vi "RemoteVI Read Tips.vi"(0 "VI":refnum<vi>, 1 "refresh?":bool, 2 "origin":cluster{"x":i32, "y":i32}, 3 "message in":string="tips []", 5 "subpanels?":bool=TRUE) -> (4 "message out":string, 15 "error out":errorcluster)   [LabVIEW 2020, in "RemoteVI.lvlib"]
doc: "Reads the tip strips of the published panel for the tips message (docs\\protocol.md 3.3) - LabVIEW shows its own tip strips only while it is the foreground application, so the browser shows them itself. When refresh? is TRUE (the server loop just refreshed the geometry: every 500 ms, never while a popup or a modal window is open, because this is a VI Server call that would block in their modal loop), every visible control with a tip strip gives one entry: the controls RemoteVI Panel Controls.vi finds (top level of every pane, the selected page of a tab control, cluster elements, two levels deep) and those of a VI shown in a subpanel among them. An entry's bounds are the control's Position and Bounds (the label included) converted from its pane's coordinates to panel coordinates ({LV.Pane} CvtPaneToPanelCoords on the pane RemoteVI Panel Controls.vi gives; a subpanel VI's panes convert into the host panel), then to screen coordinates (CvtPanelToScreenCoords of the published panel), then to frame coordinates (minus the top-left of Front Panel Window:Panel Bounds, plus origin). Inner controls come first (subpanel VIs, then deeper levels), so the browser, which shows the first entry under the pointer, shows a cluster element's tip strip rather than its cluster's. RemoteVI Tips Message.vi builds message out from them. Otherwise, or on an error, message out is message in."
uses:
  RemoteVI.lvlib
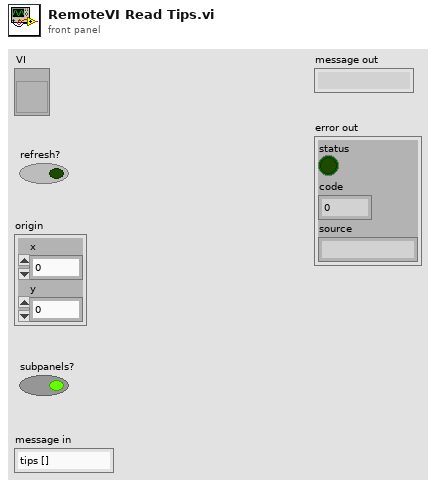
[diagram p1: front panel]
types:
  T1 = cluster{"x":i32, "y":i32, "w":i32, "h":i32, "text":string}
  T2 = typedef "LVRectTypeDef.ctl" = cluster{"left":i16, "top":i16, "right":i16, "bottom":i16}
  T3 = typedef "LVPositionTypeDef.ctl" = cluster{"Left":i32, "Top":i32}
  T4 = typedef "LVBoundsTypeDef.ctl" = cluster{"Width":u32, "Height":u32}
  T5 = typedef "LVPointTypeDef.ctl" = cluster{"Horizontal":i16, "Vertical":i16}
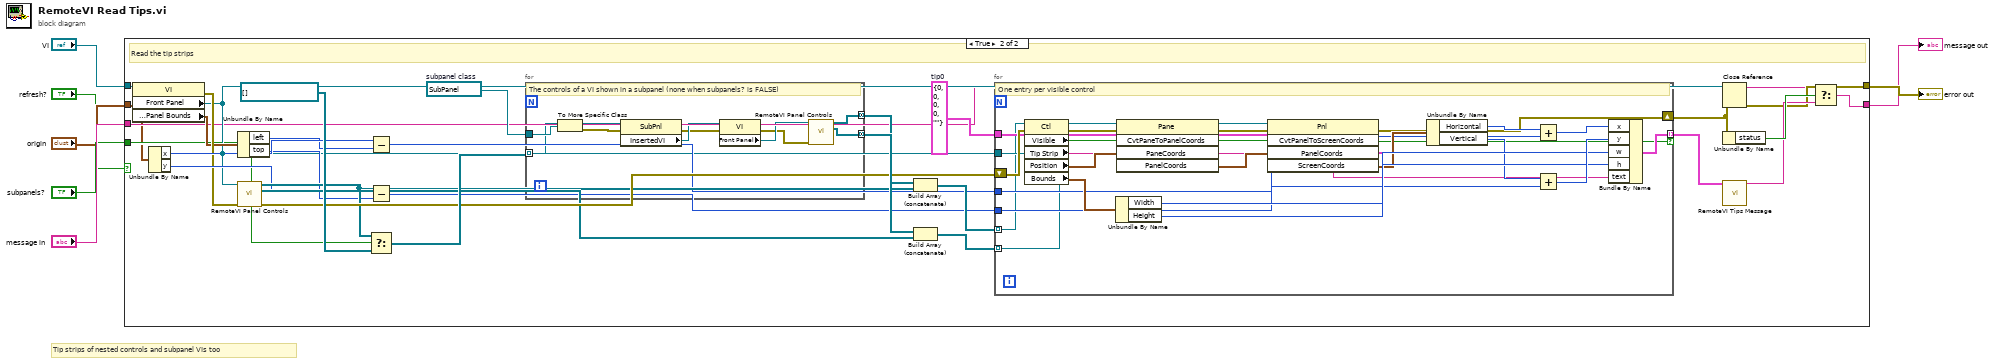
[diagram p0: block diagram]
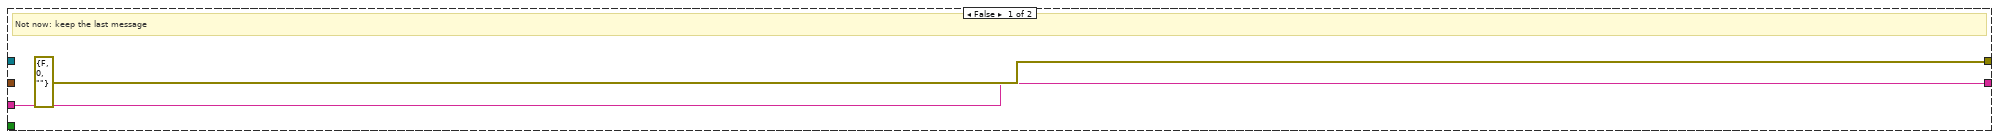
[diagram p2: hidden frame]
diagram:
  # "Tip strips of nested controls and subpanel VIs too"
  n1 = case shown="True" "refresh?" {
    tunnel: "VI" -> [_ w10]
    tunnel: "origin" -> [_ w11]
    tunnel: "message in" -> [w8 w12]
    tunnel: "subpanels?" -> [_ w13]
    tunnel: [errorcluster {"status"=FALSE, "code"=0, "source"=""} w36] -> w7
    tunnel: [w8 w39] -> w6
    frame False {
      # "Not now: keep the last message"
    }
    frame True {
      w33 = T1 {"x"=0, "y"=0, "w"=0, "h"=0, "text"=""}  # tip0
      w28 = refnum<vi> refnum  # subpanel class
      # "Read the tip strips"
      n2 = property class="VI"(reference=w10) -> (error out=w16:errorcluster, "Front Panel"=w14:refnum<vi>, "Front Panel Window:Panel Bounds"=w15:T2)  [unwired: 1 in, 1 out]
      n3 = Unbundle By Name(w11) -> ("x"=w19:i32, "y"=w20:i32)
      n4 = Unbundle By Name(w15) -> ("left"=w17:i16, "top"=w18:i16)
      n5 = call "RemoteVI Panel Controls.vi"("Panel"=w14, "error in"=w16) -> ("Controls"=w23:refnum<vi>[], "Panes"=w24:refnum<vi>[], "error out"=w25:errorcluster)  [unwired: 11 in]
      n6 = Subtract(x=w19, y=w17) -> (x-y=w21:i32)
      n7 = Subtract(x=w20, y=w18) -> (x-y=w22:i32)
      n8 = Select(t=w23, s=w13, f=refnum<vi>[] []) -> (s? t:f=w27:refnum<vi>[])
      n9 = for {
        tunnel: w28 -> [w64]
        tunnel: w27 -> [w63] mode=indexing
        tunnel: [w71] -> w29 mode=concatenating
        tunnel: [w72] -> w30 mode=concatenating
        # "The controls of a VI shown in a subpanel (none when subpanels? is FALSE)"
        n10 = To More Specific Class(target class=w64, reference=w63) -> (specific class reference=w65:refnum<vi>, error out=w66:errorcluster)  [unwired: 1 in]
        n11 = property class="SubPnl"(reference=w65, error in=w66) -> (error out=w67:errorcluster, "InsertedVI"=w68:refnum<vi>)  [unwired: 1 out]
        n12 = property class="VI"(reference=w68, error in=w67) -> (error out=w69:errorcluster, "Front Panel"=w70:refnum<vi>)  [unwired: 1 out]
        n13 = call "RemoteVI Panel Controls.vi"("Panel"=w70, "error in"=w69) -> ("Controls"=w71:refnum<vi>[], "Panes"=w72:refnum<vi>[])  [unwired: 11 in, 1 out]
      }
      n14 = Build Array (concatenate)(w29, w23) -> (w31:refnum<vi>[])
      n15 = Build Array (concatenate)(w30, w24) -> (w32:refnum<vi>[])
      n16 = for {
        tunnel: w33 -> [w44]
        tunnel: w14 -> [w45]
        shift-right: [w47] -> w34
        shift-left: w25 -> [w46]
        tunnel: w21 -> [w42]
        tunnel: w22 -> [w43]
        tunnel: w31 -> [w40] mode=indexing
        tunnel: w32 -> [w41] mode=indexing
        tunnel: [w62] -> w35 mode=indexing if=w48
        # "One entry per visible control"
        n17 = property class="Ctl"(reference=w40, error in=w46) -> (error out=w52:errorcluster, "Visible"=w48:bool, "Tip Strip"=w49:string, "Position"=w50:T3, "Bounds"=w51:T4)  [unwired: 1 out]
        n18 = Unbundle By Name(w51) -> ("Width"=w58:u32, "Height"=w59:u32)
        n19 = invoke class="Pane" method="CvtPaneToPanelCoords"(reference=w41, error in=w52, "PaneCoords"=w50) -> (error out=w53:errorcluster, "PanelCoords"=w54:T5)  [unwired: 2 in, 3 out]
        n20 = invoke class="Pnl" method="CvtPanelToScreenCoords"(reference=w45, error in=w53, "PanelCoords"=w54) -> (error out=w47:errorcluster, "ScreenCoords"=w55:T5)  [unwired: 2 in, 3 out]
        n21 = Unbundle By Name(w55) -> ("Horizontal"=w56:i16, "Vertical"=w57:i16)
        n22 = Add(x=w56, y=w42) -> (x+y=w60:i32)
        n23 = Add(x=w57, y=w43) -> (x+y=w61:i32)
        n24 = Bundle By Name(cluster=w44, "x"=w60, "y"=w61, "w"=w58, "h"=w59, "text"=w49) -> (w62:T1)
      }
      n25 = Close Reference(reference=w14, error in (no error)=w34) -> (error out=w36:errorcluster)
      n26 = Unbundle By Name(w34) -> ("status"=w38:bool)
      n27 = call "RemoteVI Tips Message.vi"("tips"=w35) -> ("message"=w37:string)  [unwired: 14 in]
      n28 = Select(t=w12, s=w38, f=w37) -> (s? t:f=w39:string)
    }
  }
  "message out" <- w6
  "error out" <- w7
